vi "Refresh Role.vi"(8 "error in (no error)":errorcluster, 11 "PluginGUI in":refnum<class "PluginGUI.lvclass">) -> (0 "error out":errorcluster, 3 "PluginGUI out":refnum<class "PluginGUI.lvclass">)   [LabVIEW 2020, in "VolatusGUI.lvlib" / "PluginGUI.lvclass"]
uses:
  PluginGUI.lvclass
  PluginGUI.lvclass/PluginGUI.ctl
  Volatus/Roles API/Roles API.lvclass/Roles API.ctl
  GUI Element/GUI Element.lvclass
  Volatus/Roles API/Roles API.lvclass
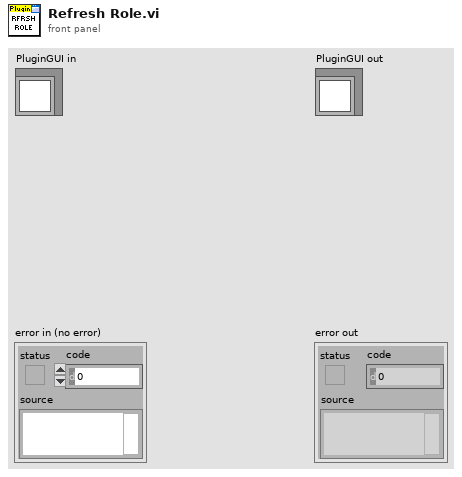
[diagram p1: front panel]
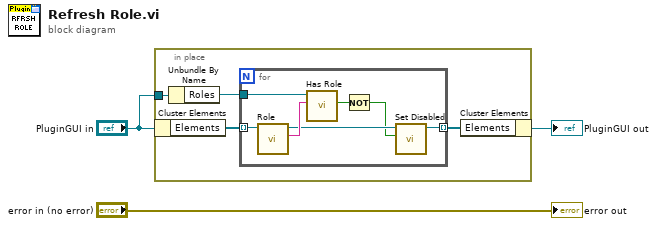
[diagram p0: block diagram]
diagram:
  n1 = in-place {
    in-place-border: "PluginGUI in" -> [w7]
    n2 = in-place-cluster #1("PluginGUI in") -> ("Elements"=w5:refnum<class "GUI Element.lvclass">[])
    n3 = Unbundle By Name(w7) -> ("Roles"=w6:refnum<class "Roles API.lvclass">)
    n4 = for {
      tunnel: w6 -> [w14]
      tunnel: [w11] -> w4 mode=indexing
      tunnel: w5 -> [w10] mode=indexing
      n5 = call "Role.vi"("GUI Element in"=w10) -> ("Role"=w13:string, "GUI Element out"=w12:refnum<class "GUI Element.lvclass">)  [unwired: 9 in]
      n6 = call "Has Role.vi"("Role"=w13, "Roles API in"=w14) -> ("Has Role"=w9:bool)  [unwired: 7 in, 2 out]
      n7 = Not(x=w9) -> (.not. x?=w8:bool)
      n8 = call-dynamic "Set Disabled.vi"("Disabled"=w8, "GUI Element in"=w12) -> ("GUI Element out"=w11:refnum<class "GUI Element.lvclass">)  [unwired: 8 in, 1 out]
    }
    n9 = in-place-cluster #1("Elements"=w4) -> (→"PluginGUI out":refnum<class "PluginGUI.lvclass">)
  }
  "error out" <- "error in (no error)"
